vi "TestOpenCycle.vi"() -> ()   [LabVIEW 2023]
uses:
  S7Plc.ctl
  D:/Projects/S7View/S7Lib/bin/Debug/S7.Net.dll
  S7Lib/bin/Debug/S7.Net.dll
panel:
  out "value":sgl
  out "S7PLC 2":T1={"ip"="192.168.10.10", "type"=40, "rack"=0, "slot"=0, "link"=FALSE, "status"=FALSE, "msg"="", "_msg"="", "plc"=refnum} caption="S7PLC" {"type" items=["S7200"=0, "Logo0BA8"=1, "S7200Smart"=2, "S7300"=10, "S7400"=20, "S71200"=30, "S71500"=40]}
  in  "等待时间（毫秒）":u32
  in  "布尔":bool
  out "S7PLC":T1={"ip"="192.168.10.10", "type"=40, "rack"=0, "slot"=0, "link"=FALSE, "status"=FALSE, "msg"="", "_msg"="", "plc"=refnum} {"type" items=["S7200"=0, "Logo0BA8"=1, "S7200Smart"=2, "S7300"=10, "S7400"=20, "S71200"=30, "S71500"=40]}
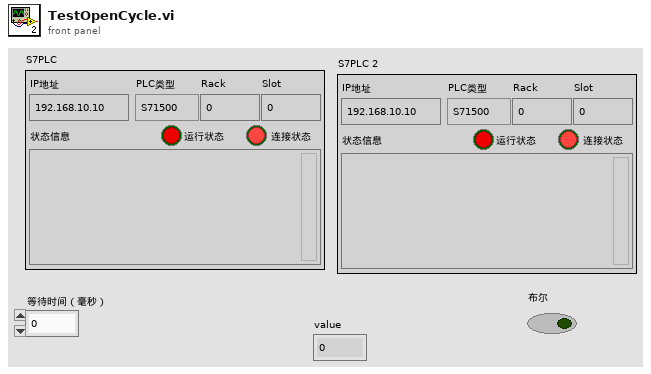
[diagram p1: front panel]
types:
  T1 = typedef "S7Plc.ctl" = cluster{"ip":string, "type":i16, "rack":i16, "slot":i16, "link":bool, "status":bool, "msg":string, "_msg":string, "plc":refnum<k24>}
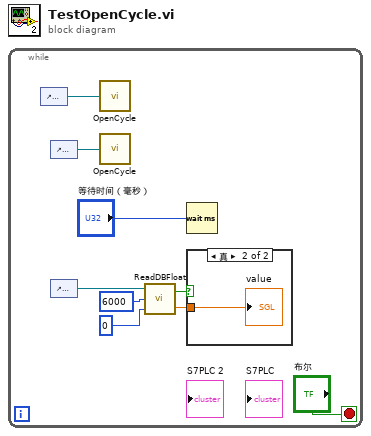
[diagram p0: block diagram]
diagram:
  n1 = while {
    stop <- "布尔" stop-if-true
    n2 = control-ref of="S7PLC 2"() -> (w2:refnum<vi>)
    n3 = control-ref of="S7PLC"() -> (w3:refnum<vi>)
    n4 = control-ref of="S7PLC"() -> (w1:refnum<vi>)
    n5 = call "OpenCycle.vi"("PLC"=w2) -> ()
    n6 = call "OpenCycle.vi"("PLC"=w3) -> ()
    n7 = call "ReadDBFloat.vi"("start"=0, "db"=6000, "PLC"=w1) -> ("value"=w5:sgl, "ok"=w4:bool)
    n8 = Wait (ms)(milliseconds to wait="等待时间（毫秒）") -> ()  [unwired: 1 out]
    n9 = case shown="真" w4 {
      tunnel: w5 -> [_ w10]
      frame False {
      }
      frame True {
        "value" <- w10
      }
    }
  }
